vi "Edit Property In Translation.vi"(7 "Languages":cluster{"ANSI":string[], "Unicode":string[]}, 8 "Property_Language":string, 9 "Translations Text":string, 10 "Control Label Name":string, 11 "Translastions in":map{string, T1}(c390)) -> (3 "Translastions out":map{string, T1}(c390))   [LabVIEW 2019, in "Language Editor.lvlib"]
doc: "- - -\nCopyright (c) 2026, Merecs Engineering GmbH"
uses:
  Language Editor.lvlib
  type defs/Cluster Translations.ctl
  Language Selection/TypeDefs/Cluster PropertyTranslation.ctl
  Language Selection/TypeDefs/Enum Property Type.ctl
  Language Selection/Language Selection.lvlib
panel:
  # "Connector Pane"
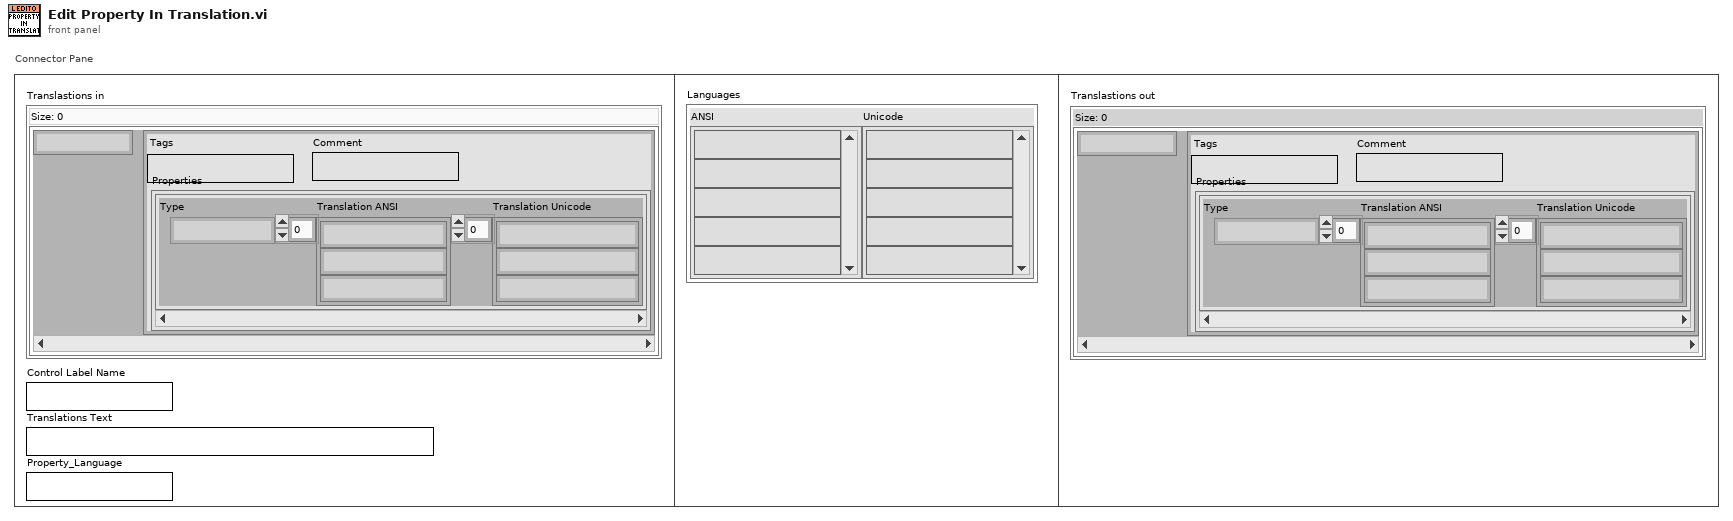
[diagram p1: front panel]
types:
  T1 = typedef "Language Editor.lvlib/Cluster Translations.ctl" = cluster{"Tags":string, "Comment":string, "Properties":T2[]}
  T2 = typedef "Language Selection.lvlib/Cluster PropertyTranslation.ctl" = cluster{"Type":T3, "Translation ANSI":string[], "Translation Unicode":string[]}
  T3 = typedef "Language Selection.lvlib/Enum Property Type.ctl" = enum16{"NA", "Caption", "String Value", "Boolean Text", "Ring Strings", "1D Array Elements", "2D Array Elements", "(MC)Listbox Header", "(MC)Listbox Items", "Tab Pages Names", "X & Y GraphChart", "Plot Names", "Table Headers", "Table Items", "TipStrip", "Combobox Strings", "Cursor Name", "Tree Col Headers"}
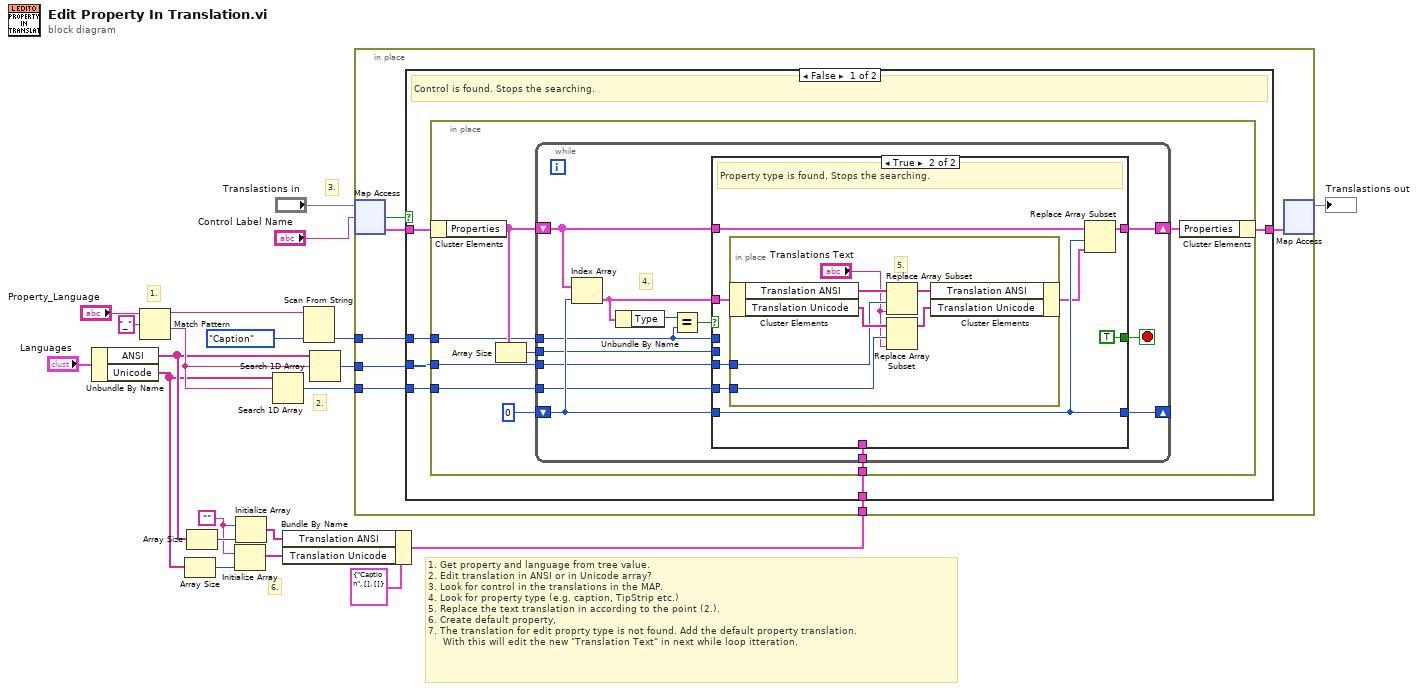
[diagram p0: block diagram]
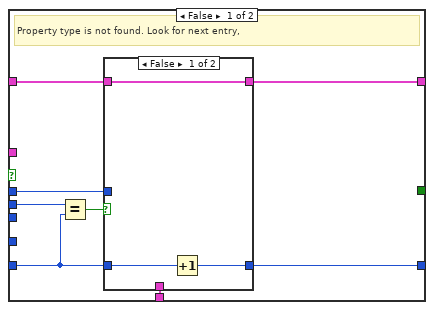
[diagram p2: hidden frame]
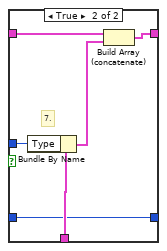
[diagram p3: hidden frame]
diagram:
  w12 = ""
  # "3."
  # "6."
  # "1."
  # "2."
  # "1. Get property and language from tree value.\n2. Edit translation in ANSI or in Unicode array?\n3. Look for control in the translations in the MAP.\n4. Look for property type (e.g. caption, TipStrip etc.)\n5. Replace the text translation in according to the point (2.).\n6. Create default property,\n7. The translation for edit proprty type is not found. Add the default property translation.\n     With this will edit the new \"Translation Text\" in next while loop itteration."
  n1 = Unbundle By Name("Languages") -> ("ANSI"=w16:string[], "Unicode"=w15:string[])
  n2 = Match Pattern(string="Property_Language", regular expression="_") -> (before substring=w18:string, after substring=w19:string)  [unwired: 1 in, 2 out]
  n3 = Array Size(array=w15) -> (size(s)=w13:i32)
  n4 = Array Size(array=w16) -> (size(s)=w14:i32)
  n5 = Initialize Array(w12, w13) -> (w9:string[])
  n6 = Initialize Array(w12, w14) -> (w10:string[])
  n7 = Search 1D Array(1D array=w15, element=w19) -> (index of element=w3:i32)  [unwired: 1 in]
  n8 = Bundle By Name(cluster=T2 {"Type"=enum."Caption", "Translation ANSI"=[], "Translation Unicode"=[]} ("Obj."), "Translation ANSI"=w10, "Translation Unicode"=w9) -> (w2:T2)
  n9 = Scan From String(input string=w18, default 1=Enum_Property_Type."Caption" ("Type")) -> (output 1=w5:T3)  [unwired: 3 in, 3 out]
  n10 = Search 1D Array(1D array=w16, element=w19) -> (index of element=w4:i32)  [unwired: 1 in]
  n11 = in-place {
    in-place-border: w5 -> [w28]
    in-place-border: w3 -> [w27]
    in-place-border: w4 -> [w26]
    in-place-border: w2 -> [w25]
    n12 = in-place-map #1("Translastions in", "Control Label Name") -> (w23:T1, w24:bool)  [unwired: 1 in]
    n13 = case shown="False" w24 {
      tunnel: [w29 w88] -> w22
      tunnel: w23 -> [w30 w88]
      tunnel: w28 -> [w34 _]
      tunnel: w26 -> [w33 _]
      tunnel: w27 -> [w32 _]
      tunnel: w25 -> [w31 _]
      frame False {
        # "Control is found. Stops the searching."
        n14 = in-place {
          in-place-border: w34 -> [w41]
          in-place-border: w33 -> [w40]
          in-place-border: w32 -> [w39]
          in-place-border: w31 -> [w36]
          n15 = in-place-cluster #2(w30) -> ("Properties"=w42:T2[])
          n16 = Array Size(array=w42) -> (size(s)=w37:i32)
          n17 = while {
            shift-right: [w49] -> w38
            shift-left: w42 -> [w54]
            tunnel: w41 -> [w45]
            tunnel: w40 -> [w53]
            tunnel: w39 -> [w52]
            tunnel: w37 -> [w44]
            tunnel: w36 -> [w48]
            shift-right: [w46] -> _
            shift-left: 0 -> [w55]
            stop <- w51 stop-if-true
            # "4."
            n18 = Index Array(array=w54, index=w55) -> (element=w50:T2)
            n19 = Unbundle By Name(w50) -> ("Type"=w47:T3)
            n20 = Equal?(x=w47, y=w45) -> (x = y?=w43:bool)
            n21 = case shown="True" w43 {
              tunnel: w50 -> [_ w79]
              tunnel: w53 -> [_ w78]
              tunnel: w52 -> [_ w77]
              tunnel: [_ TRUE] -> w51
              tunnel: w54 -> [w60 w75]
              tunnel: w55 -> [w57 w80]
              tunnel: [w61 w73] -> w49
              tunnel: w44 -> [w62 _]
              tunnel: w48 -> [w59 _]
              tunnel: [w58 w80] -> w46
              tunnel: w45 -> [w56 _]
              frame False {
                # "Property type is not found. Look for next entry,"
                n22 = Equal?(x=w62, y=w57) -> (x = y?=w63:bool)
                n23 = case shown="False" w63 {
                  tunnel: [w66 w71] -> w61
                  tunnel: w60 -> [w66 w72]
                  tunnel: w59 -> [_ w70]
                  tunnel: w56 -> [_ w68]
                  tunnel: w57 -> [w65 w67]
                  tunnel: [w64 w67] -> w58
                  frame False {
                    n24 = Increment(x=w65) -> (x+1=w64:i32)
                  }
                  frame True {
                    # "7."
                    n25 = Bundle By Name(cluster=w70, "Type"=w68) -> (w69:T2)
                    n26 = Build Array (concatenate)(w72, w69) -> (w71:T2[])
                  }
                }
              }
              frame True {
                # "Property type is found. Stops the searching."
                n27 = in-place {
                  in-place-border: w78 -> [w83]
                  in-place-border: w77 -> [w82]
                  # "5."
                  n28 = in-place-cluster #3(w79) -> ("Translation ANSI"=w87:string[], "Translation Unicode"=w85:string[])
                  n29 = Replace Array Subset(array=w87, new element="Translations Text", index=w83) -> (w86:string[])
                  n30 = Replace Array Subset(array=w85, new element="Translations Text", index=w82) -> (w84:string[])
                  n31 = in-place-cluster #3("Translation ANSI"=w86, "Translation Unicode"=w84) -> (w74:T2)
                }
                n32 = Replace Array Subset(array=w75, new element=w74, index=w80) -> (w73:T2[])
              }
            }
          }
          n33 = in-place-cluster #2("Properties"=w38) -> (w29:T1)
        }
      }
      frame True {
        # "Control not found. Look for next entry."
      }
    }
    n34 = in-place-map #1(w22) -> (→"Translastions out":map{string, T1})  [unwired: 1 in, 2 out]
  }
